vi "Host Main.vi"() -> ()   [LabVIEW 2017]
doc: "This application launches and executes the Tag Bus Data framework configuration for the specified target alias. This is a simple example of the framework API functions, but may also be a suitable starting point for a Host UI or Thick Client that is running a local version of the framework."
uses:
  <vilib>/NI/Module Execution Interface/Engine Runtime/Execution States.ctl
  <vilib>/NI/Module Execution Interface/Engine Runtime/Fault.ctl
  <vilib>/NI/Tag Bus Module Framework/runtime/error classification.ctl
  Utilities/Controlword_Commands.ctl
  Utilities/StateMachine.ctl
  module/execution/parameter user data.ctl
  <vilib>/NI/STM/TCP/TCP Read Options.ctl
  <vilib>/NI/STM/TCP/Read Meta Data (TCP Ref).vi
  <vilib>/NI/STM/TCP/Get Connection Reference (TCP).vi
  <vilib>/NI/STM/TCP/Read Meta Data (TCP Clst).vi
  <vilib>/NI/STM/Connection Manager/TCP/TCP Connection Manager.vi
  <vilib>/NI/STM/TCP/Write Message (TCP).vi
  <vilib>/NI/STM/TCP/Read Message (TCP).vi
  <vilib>/userdefined/High Color/nirio_resource_hc.ctl
  <vilib>/NI/Module Execution Interface/Engine Runtime/Engine Runtime Interface.lvclass
  <vilib>/NI/DCAF/Tag Editor Core/Framework Configuration Classes/target runtime/PL_Target Runtime.lvclass
  <vilib>/NI/Tag Bus Module Framework/FPGA manager/FPGA manager.lvlib
  <vilib>/rvi/interface/nirviOpenFPGA/nirviOpenFPGA.xnode
  <vilib>/NI/Tag Bus Module Framework/FPGA manager/methods.ctl
  <vilib>/NI/Tag Bus Module Framework/runtime/TBM module execution interface.lvclass
  <vilib>/NI/STM/NI STM.lvlib
  Utilities/WordManipulationLibrary.lvlib
  module/execution/ExampleSequencer runtime.lvclass
panel:
  in  "Velocity Move":bool
  out "Results":dbl[](array[numeric])
  out "Status":T1
  in  "Positions":dbl[](array[numeric])
  in  "Velocity":dbl=1000.0
  in  "Acceleration":dbl=10000.0
  in  "Acceleration Jerk":dbl=1000.0
  in  "StraightLineMove":bool
  in  "StateChange":bool
  in  "Device Control Command":T2
  in  "StateName":string="StateChange"
  in  "Target IP Address":string="localhost"
  in  "Network Stop":bool
  out "error  out":errorcluster
  in  "configuration file path":path
  in  "target alias":string="PC"
  out "engine status":T6(array[cluster])
  in  "Engine_Stop":bool
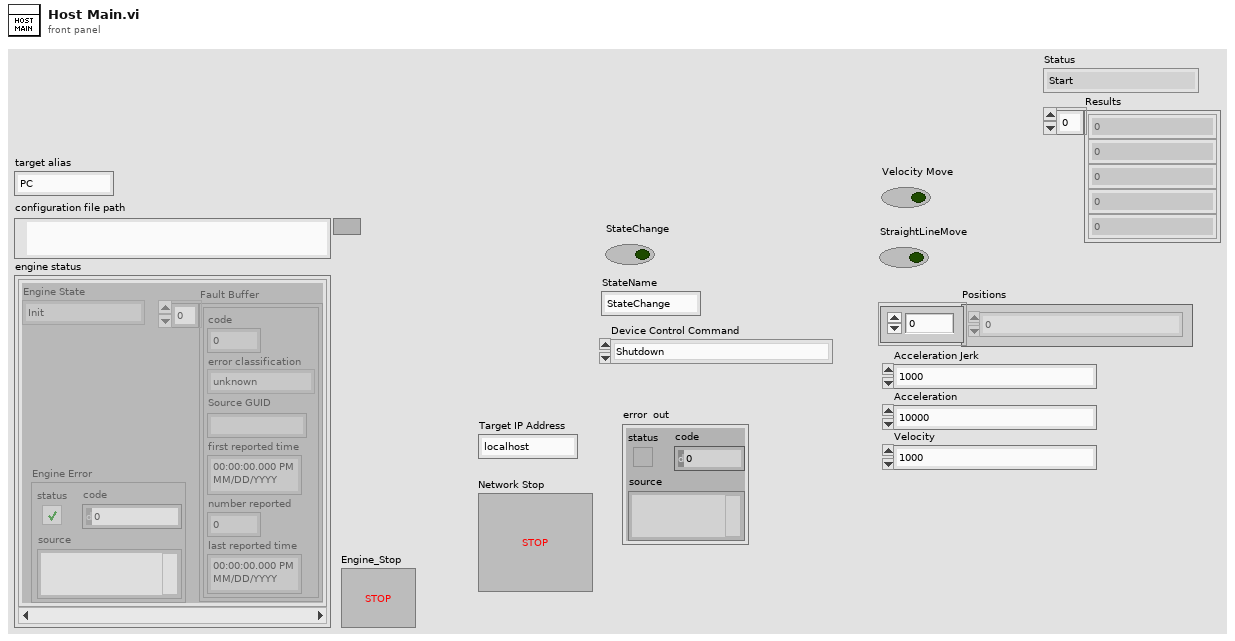
[diagram p1: front panel]
types:
  T1 = typedef "WordManipulationLibrary.lvlib/StateMachine.ctl" = enum16{"Start", "Not Ready to Switch On", "Switch On Disabled", "Ready to Switch On", "Switched On", "Operation enable", "Quick Stop Active", "Fault Reaction Active", "Fault"}
  T2 = typedef "WordManipulationLibrary.lvlib/Controlword_Commands.ctl" = enum16{"Shutdown", "Switch On", "Disable Voltage", "Quick Stop", "Disable Op", "Enable Op", "Fault Reset", "Error"}
  T3 = typedef "Engine Runtime Interface.lvclass/Execution States.ctl" = enum16{"Init", "Pre-Operational", "Safe-Operational", "Operational", "Stopped"}
  T4 = typedef "Engine Runtime Interface.lvclass/Fault.ctl" = cluster{"code":i32, "error classification":T5, "Source GUID":string, "first reported time":timestamp, "number reported":u32, "last reported time":timestamp}
  T5 = typedef "TBM module execution interface.lvclass/error classification.ctl" = enum16{"unknown", "none", "trivial", "recoverable", "critical"}
  T6 = cluster{"Engine State":T3, "Fault Buffer":T4[], "Engine Error":errorcluster}[]
  T7 = typedef "ExampleSequencer runtime.lvclass/parameter user data.ctl" = cluster{"Statusword":u16, "Results":dbl[]}
  T8 = typedef "NI STM.lvlib/TCP Read Options.ctl" = cluster{"ignore timeout error":bool, "timeout ms (1000)":i32}
  T9 = typedef "NI STM.lvlib/TCP Connection Info.ctl" = cluster{"connection ID":refnum<k5>, "meta data":T10[]}
  T10 = typedef "NI STM.lvlib/MetaDataElement.ctl" = string
  T11 = typedef "FPGA manager.lvlib/methods.ctl" = enum16{"initialize bitfile", "cache bitfile", "locate bitfile", "close bitfile", "clear manager"}
  T12 = typedef "nirio_resource_hc.ctl" = tag
  T13 = cluster{"Engine State":T3, "Fault Buffer":T4[], "Engine Error":errorcluster}
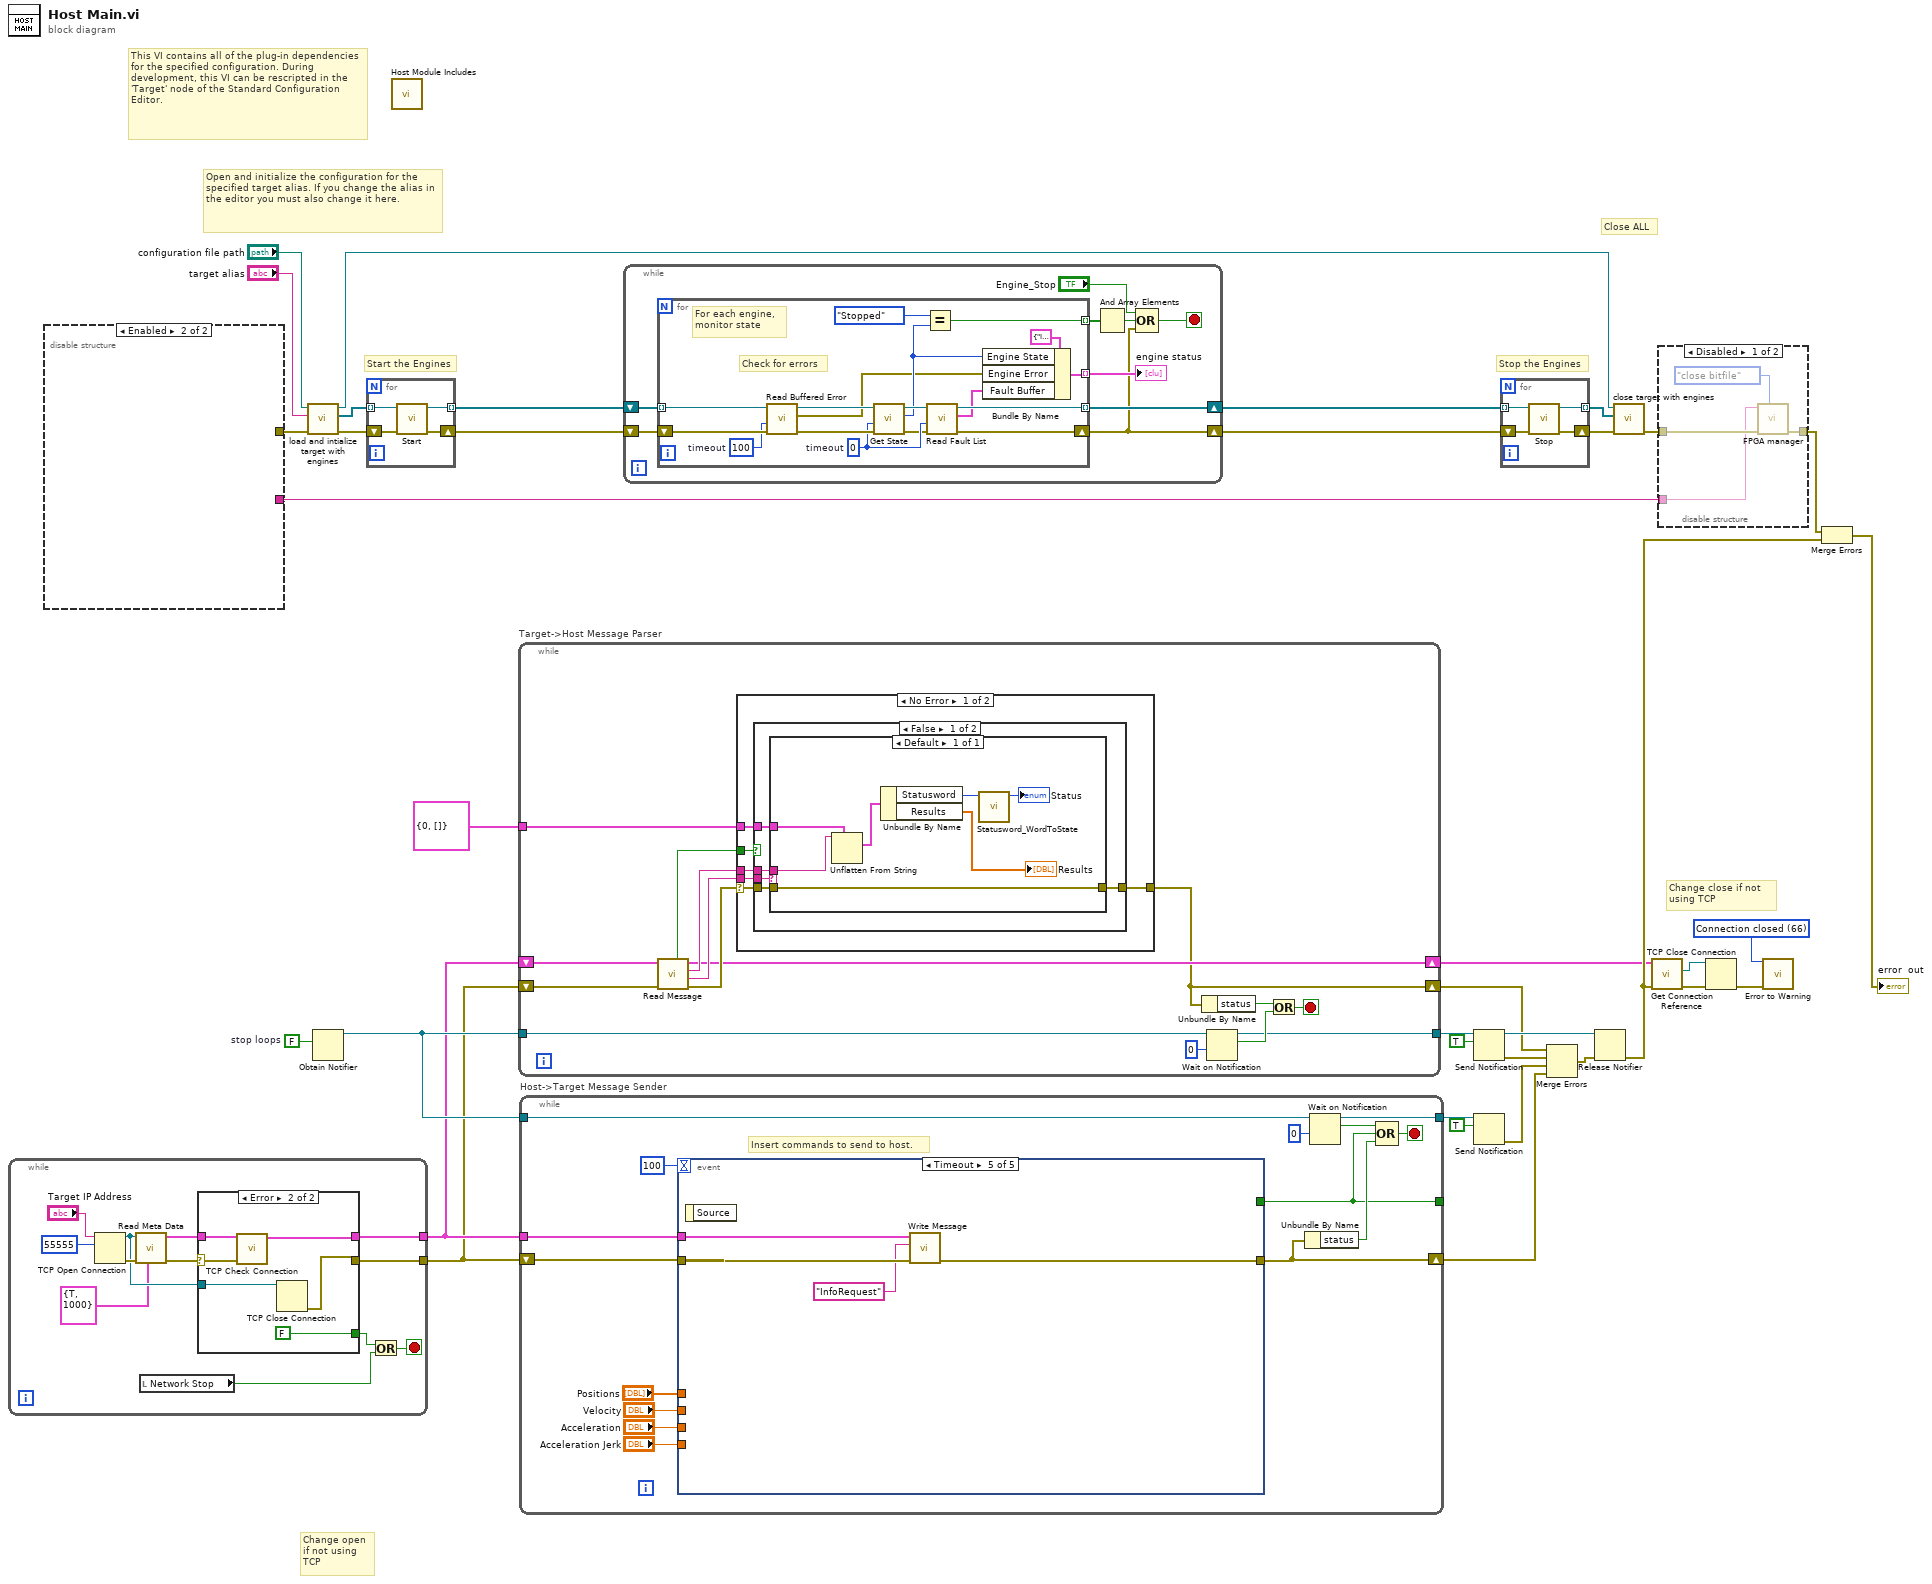
[diagram p0: block diagram]
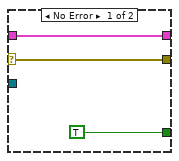
[diagram p2: hidden frame]
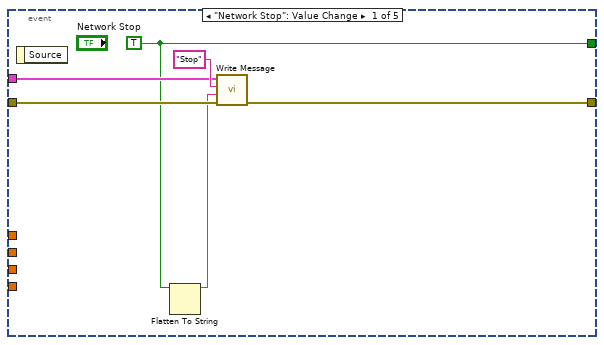
[diagram p3: hidden frame]
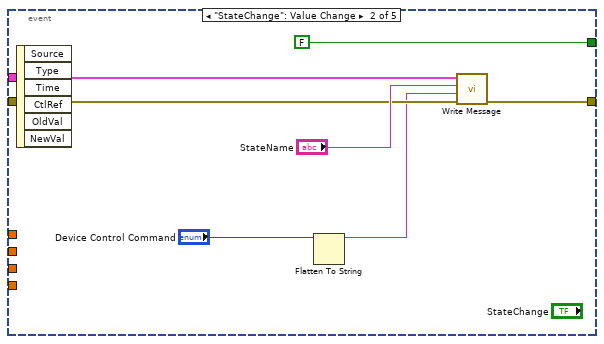
[diagram p4: hidden frame]
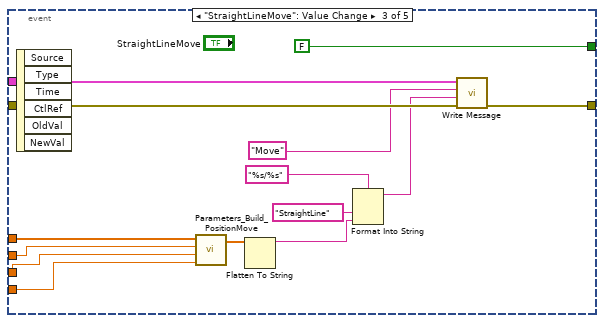
[diagram p5: hidden frame]
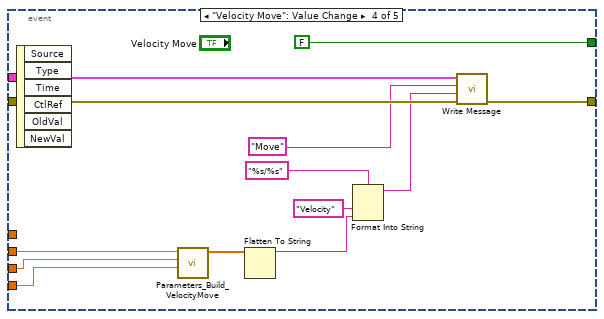
[diagram p6: hidden frame]
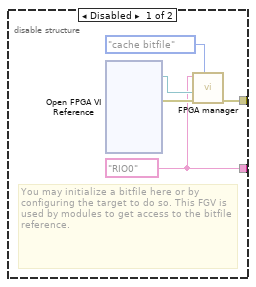
[diagram p10: hidden frame]
diagram:
  w6 = FALSE  # stop loops
  w20 = 66 items=["No Error", "Argument Error", "Memory Full", "Out of Zone", "End of File", "File Already Open", "Generic File IO Error", "File Not Found", "File Permission Error", "Disk Full", "Duplicate Path", "Too Many Files Open", "Not Enabled", "Resource File Not Found", "Cannot Add Resource", "Resource Not Found", "Image Not Found", "Image Memory Error", "Pen Does Not Exist", "Config Bad Type", "Config Token Not Found", "Config Parse Error", "Config Memory Error", "Bad External Code Format", "Bad External Code Offset", "External Code Not Present", "Null Window", "Destroy Window Mixup", "Null Menu", "Print Aborted", "Bad Print Record", "Print Driver Error", "Windows Error During Print", "Memory Error During Print", "Print Dialog Error", "Generic Print Error", "Invalid Device Refnum", "Device Not Found", "Device Parameter Error", "Device Unit Error", "Can't Open Device", "Device Call Aborted", "Generic Error", "Cancelled By User", "Object ID Too Low", "Object ID Too High", "Object Not In Heap", "Unknown Heap", "Bad DefProc ID", "DefProc Not In Table", "Message Out Of Range", "Null Method", "Unknown Message", "Manager Call Not Supported", "Bad address", "Connection In progress", "Connection timed out", "Connection is already in progress", "Network attribute not supported", "Network error", "Address in use", "System out of memory", "Connection aborted", "Connection refused", "Connection is not connected", "Connection is already connected", "Connection closed", "Initialize error (interapplication manager)", "Bad occurrence", "Wait on unbound occurrence handler", "Occurrence queue overflow", "Bad path", "Semaphore not signaled", "Unrecognized type (interapplication manager)"] ("1st Error to Convert")
  # "Change close if not using TCP"
  # "Change open if not using TCP"
  # "Start the Engines"
  # "Open and initialize the configuration for the specified target alias. If you change the alias in the editor you must also change it here."
  # "Close ALL"
  # "Stop the Engines"
  # "This VI contains all of the plug-in dependencies for the specified configuration. During development, this VI can be rescripted in the 'Target' node of the Standard Configuration Editor."
  n1 = while {
    tunnel: [w45] -> w5
    tunnel: [w43] -> w4
    stop <- w40 stop-if-true
    n2 = TCP Open Connection(address="Target IP Address", remote port or service name=u16 55555 ("remote port")) -> (connection ID=w42:refnum<k5>, error out=w49:errorcluster)  [unwired: 1 in, 2 out]
    n3 = call-poly <vilib>:"Read Meta Data.vi"("options"=T8 {"ignore timeout error"=TRUE, "timeout ms (1000)"=1000}, "error in"=w49, "connection ID"=w42) -> ("error out"=w46:errorcluster, "connection info out"=w44:T9)  [unwired: 7 out]
    n4 = local read "Network Stop"() -> (w39:bool)
    n5 = case shown="Error" w46 {
      selector: w46 -> [w50 w56]
      tunnel: [TRUE FALSE] -> w41
      tunnel: [w51 w55] -> w45
      tunnel: w44 -> [w51 w57]
      tunnel: [w50 w53] -> w43
      tunnel: w42 -> [_ w58]
      frame No Error {
      }
      frame Error {
        n6 = call <vilib>:"TCP Check Connection.vi"("error in"=w56, "connection in"=w57) -> ("connection out"=w55:T9)  [unwired: 7 in, 2 out]
        n7 = TCP Close Connection(connection ID=w58) -> (error out=w53:errorcluster)  [unwired: 2 in, 1 out]
      }
    }
    n8 = Or(x=w41, y=w39) -> (x .or. y?=w40:bool)
  }
  n9 = disable-structure shown="Enabled" {
    disable-tunnel: [w63 _] -> w27
    disable-tunnel: [w59 _] -> w26
    frame Disabled {
      w59 = T12 "RIO0" ("RIO resource")
      # "You may initialize a bitfile here or by configuring the target to do so. This FGV is used by modules to get access to the bitfile reference."
      n10 = xnode "Open FPGA VI Reference"() -> ("FPGA VI Reference Out"=w61:refnum<k20>, "error out"=w62:errorcluster)  [unwired: 2 in]
      n11 = call <vilib>:"FPGA manager.vi"("action"=methods."cache bitfile", "error in"=w62, "bitfile to cache"=w61, "RIO resource"=w59) -> ("error out"=w63:errorcluster)  [unwired: 5 in, 2 out]
    }
    frame Enabled {
    }
  }
  n12 = call <vilib>:"load and intialize target with engines.vi"("error in"=w27, "target alias"="target alias", "file path"="configuration file path") -> ("error out"=w34:errorcluster, "engine runtime interfaces"=w33:refnum<class "Engine Runtime Interface.lvclass">[], "target runtime"=w30:refnum<class "PL_Target Runtime.lvclass">)  [unwired: 6 in]
  n13 = Obtain Notifier(notification data type=w6) -> (notifier out=w9:refnum<notifier>)  [unwired: 3 in, 2 out]
  n14 = for {
    tunnel: [w67] -> w37 mode=indexing
    tunnel: w33 -> [w64] mode=indexing
    shift-right: [w66] -> w22
    shift-left: w34 -> [w65]
    n15 = call-dynamic "Start.vi"("error in"=w65, "Engine Runtime Interface in"=w64) -> ("error out"=w66:errorcluster, "Engine Runtime Interface out"=w67:refnum<class "Engine Runtime Interface.lvclass">)  [unwired: 8 in]
  }
  n16 = call "Host Module Includes.vi"() -> ()  [unwired: 12 in]
  n17 = while "Target->Host Message Parser" {
    shift-right: [w69] -> w3
    shift-left: w4 -> [w81]
    tunnel: w9 -> [w75]
    tunnel: [w71] -> w7
    shift-right: [w76] -> w19
    shift-left: w5 -> [w82]
    tunnel: T7 {"Statusword"=0, "Results"=[]} ("Parameters to process") -> [w68]
    stop <- w72 stop-if-true
    n18 = call-poly <vilib>:"Read Message.vi"("error in"=w81, "connection info in"=w82) -> ("error out"=w77:errorcluster, "name"=w80:T10, "data string"=w79:string, "connection info out"=w76:T9, "timed out?"=w78:bool)  [unwired: 3 in, 2 out]
    n19 = case shown="No Error" w77 {
      selector: w77 -> [w85 w102]
      tunnel: w80 -> [w88 _]
      tunnel: w79 -> [w87 _]
      tunnel: w78 -> [w86 _]
      tunnel: [w84 w102] -> w69
      tunnel: w68 -> [w83 _]
      frame No Error {
        n20 = case shown="False" w86 {
          tunnel: w88 -> [w90 _]
          tunnel: w87 -> [w93 _]
          tunnel: w85 -> [w92 w101]
          tunnel: [w91 w101] -> w84
          tunnel: w83 -> [w89 _]
          frame False {
            n21 = case shown="Default" w90 {
              tunnel: w93 -> [w99]
              tunnel: w92 -> [w100]
              tunnel: [w100] -> w91
              tunnel: w89 -> [w98]
              frame Default {
                n22 = Unflatten From String(type=w98, binary string=w99) -> (value=w97:T7)  [unwired: 3 in, 2 out]
                n23 = Unbundle By Name(w97) -> ("Statusword"=w96:u16, "Results"=→"Results":dbl[])
                n24 = call "Statusword_WordToState.vi"("Data_In"=w96) -> ("Status"=→"Status":T1)  [unwired: 10 in]
              }
            }
          }
          frame True {
          }
        }
      }
      frame Error {
      }
    }
    n25 = Unbundle By Name(w69) -> ("status"=w70:bool)
    n26 = Wait on Notification(notifier=w75, timeout in ms (-1)=0) -> (notifier out=w71:refnum<notifier>, notification=w73:bool)  [unwired: 2 in, 2 out]
    n27 = Or(x=w70, y=w73) -> (x .or. y?=w72:bool)
  }
  n28 = while "Host->Target Message Sender" {
    shift-right: [w109] -> w12
    shift-left: w4 -> [w117]
    tunnel: w5 -> [w116]
    tunnel: w9 -> [w113]
    tunnel: [w110] -> w10
    tunnel: [w107] -> _
    stop <- w111 stop-if-true
    # "Insert commands to send to host."
    n29 = event shown="[4] Timeout" {
      selector: _ -> [_ _ _ _ _]
      dyn-events: _ -> [_ _ _ _ _]
      timeout: 100 -> [_ _ _ _ _]
      tunnel: w116 -> [w122 w129 w144 w157 w158]
      tunnel: w117 -> [w121 w128 w143 w156 w161]
      tunnel: [w119 FALSE ("stop") FALSE ("stop") FALSE ("stop") _] -> w107
      tunnel: [w118 w125 w141 w154 w160] -> w109
      tunnel: "Positions" -> [_ _ w134 _ _]
      tunnel: "Velocity" -> [_ _ w133 w148 _]
      tunnel: "Acceleration" -> [_ _ w132 w146 _]
      tunnel: "Acceleration Jerk" -> [_ _ w131 w145 _]
      event "Network Stop": Value Change {
        w119 = TRUE ("stop")
        n30 = event-data() -> ()  [unwired: 2 out]
        n31 = Flatten To String(anything=w119) -> (data string=w120:string)  [unwired: 2 in, 3 out]
        n32 = call-poly <vilib>:"Write Message.vi"("error in"=w121, "data"=w120, "name"="Stop" ("Name"), "connection info in"=w122) -> ("error out"=w118:errorcluster)  [unwired: 1 in, 6 out]
      }
      event "StateChange": Value Change {
        n33 = event-data() -> ()  [unwired: 7 out]
        n34 = Flatten To String(anything="Device Control Command") -> (data string=w127:string)  [unwired: 2 in, 3 out]
        n35 = call-poly <vilib>:"Write Message.vi"("error in"=w128, "data"=w127, "name"="StateName", "connection info in"=w129) -> ("error out"=w125:errorcluster)  [unwired: 1 in, 6 out]
      }
      event "StraightLineMove": Value Change {
        n36 = event-data() -> ()  [unwired: 7 out]
        n37 = call "Parameters_Build_PositionMove.vi"("Acceleration Jerk"=w131, "Acceleration"=w132, "Velocity"=w133, "Positions"=w134) -> ("Parameters"=w136:dbl[])  [unwired: 7 in]
        n38 = Flatten To String(anything=w136) -> (data string=w135:string)  [unwired: 2 in, 3 out]
        n39 = Format Into String(format string="%s/%s", "StraightLine" ("input 1"), w135) -> (resulting string=w137:string)  [unwired: 2 in, 1 out]
        n40 = call-poly <vilib>:"Write Message.vi"("error in"=w143, "data"=w137, "name"="Move", "connection info in"=w144) -> ("error out"=w141:errorcluster)  [unwired: 1 in, 6 out]
      }
      event "Velocity Move": Value Change {
        n41 = event-data() -> ()  [unwired: 7 out]
        n42 = call "Parameters_Build_VelocityMove.vi"("Acceleration Jerk"=w145, "Acceleration"=w146, "Velocity"=w148) -> ("Parameters"=w147:dbl[])  [unwired: 8 in]
        n43 = Flatten To String(anything=w147) -> (data string=w149:string)  [unwired: 2 in, 3 out]
        n44 = Format Into String(format string="%s/%s", "Velocity" ("input 1"), w149) -> (resulting string=w150:string)  [unwired: 2 in, 1 out]
        n45 = call-poly <vilib>:"Write Message.vi"("error in"=w156, "data"=w150, "name"="Move", "connection info in"=w157) -> ("error out"=w154:errorcluster)  [unwired: 1 in, 6 out]
      }
      event Timeout {
        n46 = event-data() -> ()  [unwired: 2 out]
        n47 = call-poly <vilib>:"Write Message.vi"("error in"=w161, "name"="InfoRequest", "connection info in"=w158) -> ("error out"=w160:errorcluster)  [unwired: 7 in, 1 out]
      }
    }
    n48 = Unbundle By Name(w109) -> ("status"=w108:bool)
    n49 = Wait on Notification(notifier=w113, timeout in ms (-1)=0) -> (notifier out=w110:refnum<notifier>, notification=w115:bool)  [unwired: 2 in, 2 out]
    n50 = Compound Arithmetic op=OR(w115, w107, w108) -> (w111:bool)
  }
  n51 = while {
    shift-right: [w168] -> w36
    shift-left: w37 -> [w170]
    shift-right: [w162] -> w35
    shift-left: w22 -> [w169]
    stop <- w166 stop-if-true
    n52 = for {
      tunnel: w170 -> [w187] mode=indexing
      tunnel: [w179] -> w168 mode=indexing
      tunnel: [w182] -> w164 mode=indexing
      shift-right: [w178] -> w162
      shift-left: w169 -> [w186]
      tunnel: [w174] -> w165 mode=indexing
      w177 = 0  # timeout
      w181 = 100  # timeout
      # "For each engine, \nmonitor state"
      # "Check for errors"
      n53 = call-dynamic "Read Buffered Error.vi"("error in"=w186, "timeout in ms (0)"=w181, "Engine Runtime Interface in"=w187) -> ("error out"=w184:errorcluster, "Engine Error"=w172:errorcluster, "Engine Runtime Interface out"=w185:refnum<class "Engine Runtime Interface.lvclass">)  [unwired: 6 in]
      n54 = call-dynamic "Get State.vi"("error in"=w184, "timeout (-1)"=w177, "Engine Runtime Interface in"=w185) -> ("error out"=w171:errorcluster, "Engine State"=w176:T3, "Engine Runtime Interface out"=w180:refnum<class "Engine Runtime Interface.lvclass">)  [unwired: 6 in]
      n55 = Equal?(x=Execution_States."Stopped" ("Engine State"), y=w176) -> (x = y?=w182:bool)
      n56 = call-dynamic "Read Fault List.vi"("error in"=w171, "timeout (-1)"=w177, "Engine Runtime Interface in"=w180) -> ("error out"=w178:errorcluster, "faults"=w175:T4[], "Engine Runtime Interface out"=w179:refnum<class "Engine Runtime Interface.lvclass">)  [unwired: 6 in]
      n57 = Bundle By Name(cluster=T13 {"Engine State"=enum."Init", "Fault Buffer"=[], "Engine Error"={"status"=FALSE, "code"=0, "source"=""}}, "Engine State"=w176, "Engine Error"=w172, "Fault Buffer"=w175) -> (w174:T13)
    }
    "engine status" <- w165
    n58 = And Array Elements(Boolean array=w164) -> (logical AND=w163:bool)
    n59 = Compound Arithmetic op=OR("Engine_Stop", w163, w162) -> (w166:bool)
  }
  n60 = Send Notification(notification=TRUE, notifier=w7) -> (notifier out=w15:refnum<notifier>, error out=w14:errorcluster)  [unwired: 1 in]
  n61 = Send Notification(notification=TRUE, notifier=w10) -> (error out=w13:errorcluster)  [unwired: 1 in, 1 out]
  n62 = for {
    tunnel: w36 -> [w191] mode=indexing
    shift-right: [w188] -> w29
    shift-left: w35 -> [w190]
    tunnel: [w189] -> w31 mode=indexing
    n63 = call-dynamic "Stop.vi"("error in"=w190, "Engine Runtime Interface in"=w191) -> ("error out"=w188:errorcluster, "Engine Runtime Interface out"=w189:refnum<class "Engine Runtime Interface.lvclass">)  [unwired: 8 in]
  }
  n64 = Merge Errors(w3, w14, w13, w12) -> (w16:errorcluster)
  n65 = Release Notifier(notifier=w15, error in (no error)=w16) -> (error out=w23:errorcluster)  [unwired: 1 in, 2 out]
  n66 = call <vilib>:"close target with engines.vi"("error in"=w29, "Engine Runtime Interfaces"=w31, "Target Runtime"=w30) -> ("error out"=w25:errorcluster)  [unwired: 8 in]
  n67 = call-poly <vilib>:"Get Connection Reference.vi"("error in"=w23, "connection info in"=w19) -> ("error out"=w18:errorcluster, "connection ID out"=w17:refnum<k5>)  [unwired: 8 out]
  n68 = disable-structure shown="Disabled" {
    disable-tunnel: [w194 w196] -> w24
    disable-tunnel: w25 -> [w195 w196]
    disable-tunnel: w26 -> [w192 _]
    frame Disabled {
      n69 = call <vilib>:"FPGA manager.vi"("action"=methods."close bitfile", "error in"=w195, "RIO resource"=w192) -> ("error out"=w194:errorcluster)  [unwired: 6 in, 2 out]
    }
    frame Enabled {
    }
  }
  n70 = TCP Close Connection(connection ID=w17, error in (no error)=w18) -> (error out=w21:errorcluster)  [unwired: 2 out]
  n71 = call <vilib>:"Error to Warning.vi"("1st Error to Convert"=w20, "error in"=w21) -> ()  [unwired: 3 in, 11 out]
  n72 = Merge Errors(w24, w23) -> (→"error  out":errorcluster)
